vi "ADB Execute.vi"(8 "Expected Response":string, 9 "Arguments":string, 10 "Device":string, 11 "ADB Path":string="C:\\Projects\\Maestro\\PLTS\\ADB\\support") -> (0 "error out":errorcluster, 2 "Successful":bool, 3 "Response":string)   [LabVIEW 2018]
uses:
  <vilib>/regexp/Match Regular Expression.xnode
panel:
  in  "Regex Expected Response":bool
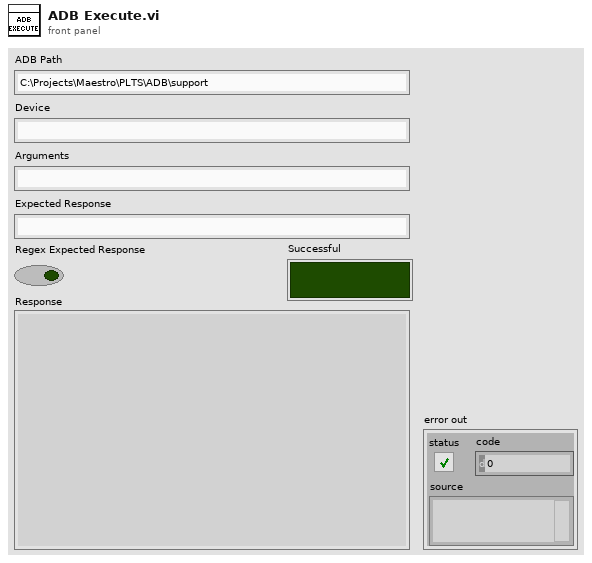
[diagram p1: front panel]
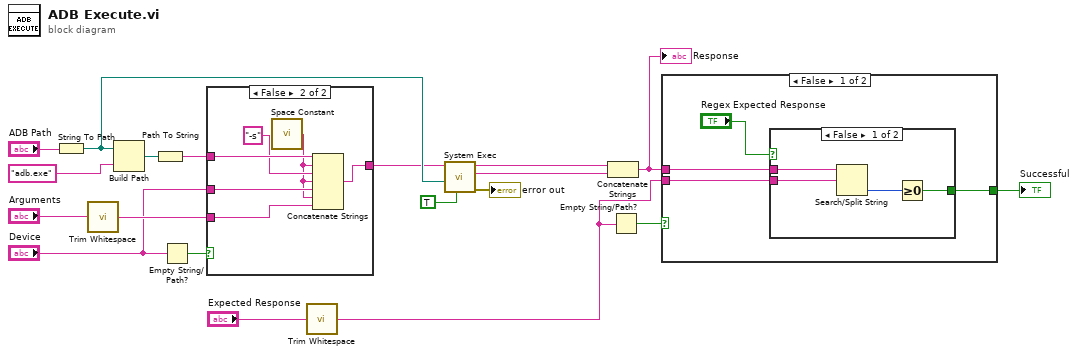
[diagram p0: block diagram]
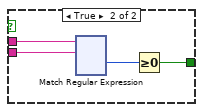
[diagram p2: hidden frame]
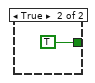
[diagram p3: hidden frame]
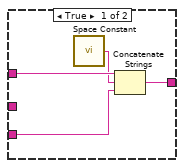
[diagram p4: hidden frame]
diagram:
  n1 = String To Path(string="ADB Path") -> (path=w17:path)
  n2 = call <vilib>:"Trim Whitespace.vi"("string"="Arguments") -> ("trimmed string"=w11:string)  [unwired: 1 in]
  n3 = Build Path(base path=w17, name or relative path="adb.exe") -> (appended path=w16:path)
  n4 = Path To String(path=w16) -> (string=w15:string)
  n5 = Empty String/Path?(string/path="Device") -> (empty?=w8:bool)
  n6 = case shown="False" w8 {
    tunnel: w15 -> [w23 w29]
    tunnel: [w22 w28] -> w14
    tunnel: w11 -> [w20 w24]
    tunnel: "Device" -> [_ w26]
    frame True {
      n7 = call <vilib>:"Space Constant.vi"() -> ("String"=w21:string)
      n8 = Concatenate Strings(w23, w21, w20) -> (w22:string)
    }
    frame False {
      n9 = call <vilib>:"Space Constant.vi"() -> ("String"=w25:string)
      n10 = Concatenate Strings(w29, w25, "-s", w25, w26, w25, w24) -> (w28:string)
    }
  }
  n11 = call <vilib>:"Trim Whitespace.vi"("string"="Expected Response") -> ("trimmed string"=w4:string)  [unwired: 1 in]
  n12 = call <vilib>:"System Exec.vi"("run minimized? (F)"=TRUE, "working directory"=w17, "command line"=w14) -> ("error out"=→"error out":errorcluster, "standard error"=w9:string, "standard output"=w10:string)  [unwired: 5 in, 1 out]
  n13 = Concatenate Strings(w10, w9) -> (w2:string)
  "Response" <- w2
  n14 = Empty String/Path?(string/path=w4) -> (empty?=w5:bool)
  n15 = case shown="False" w5 {
    tunnel: w2 -> [w33 _]
    tunnel: w4 -> [w32 _]
    tunnel: [w30 TRUE] -> w3
    frame False {
      n16 = case shown="False" "Regex Expected Response" {
        tunnel: w33 -> [w37 w40]
        tunnel: w32 -> [w36 w39]
        tunnel: [w34 w38] -> w30
        frame False {
          n17 = Search/Split String(string=w37, search string/char (-)=w36) -> (offset of match=w35:i32)  [unwired: 1 in, 2 out]
          n18 = Greater Or Equal To 0?(x=w35) -> (x >= 0?=w34:bool)
        }
        frame True {
          n19 = xnode "Match Regular Expression"("input string"=w40, "regular expression"=w39) -> ("offset past match"=w41:i32)  [unwired: 4 in, 4 out]
          n20 = Greater Or Equal To 0?(x=w41) -> (x >= 0?=w38:bool)
        }
      }
    }
    frame True {
    }
  }
  "Successful" <- w3
